vi "Test App.vi"() -> ()   [LabVIEW 2023]
uses:
  typedef/od index.ctl
  xnet_canopen.lvlib
  OD Batch.lvclass
  typedef/Runtime State.ctl
  typedef/NMT State.ctl
  typedef/canopen status formatted.ctl
  <vilib>/Utility/Data Type/Type Definitions/Data Type.ctl
  <vilib>/Utility/Data Type/NI_Data Type.lvlib
panel:
  in  "CAN Interface":refnum<k21>
  out "error out":errorcluster
  out "Write Err":string
  in  "Write Values 2":dbl[](array[numeric])
  in  "Write Values 1":dbl[](array[numeric])
  out "Read Err":string
  out "Read Values 2":T2
  out "Read Values 1":T2
  out "CANOpen Status":T3 {"NMT State" items=["Unknown"=-1, "Initializing"=0, "Pre-Operational"=127, "Operational"=5, "Stopped"=4, "?"=255]; "can_error_status" format="%.0x"}
  in  "Stop":bool
  in  "Start":bool
  in  "Write Batch 2":T6[](array[typedef]) {"SubIndex" format="%.0x"; "Index" format="%.0x"}
  in  "Write Batch 1":T6[](array[typedef]) {"SubIndex" format="%.0x"; "Index" format="%.0x"}
  in  "Read Batch 2":T6[](array[typedef]) {"SubIndex" format="%.0x"; "Index" format="%.0x"}
  in  "Read Batch 1":T6[](array[typedef]) {"SubIndex" format="%.0x"; "Index" format="%.0x"}
  in  "CANOpen LSS Persistence JSON":path
  in  "CANOpen Model JSON":path
  # "Step 1: specify model json and LSS json, \nLSS json will be created if not exists."
  # "Step 3: start if step 1 & 2 are finished."
  # "Step 2: specify Batches to read and write"
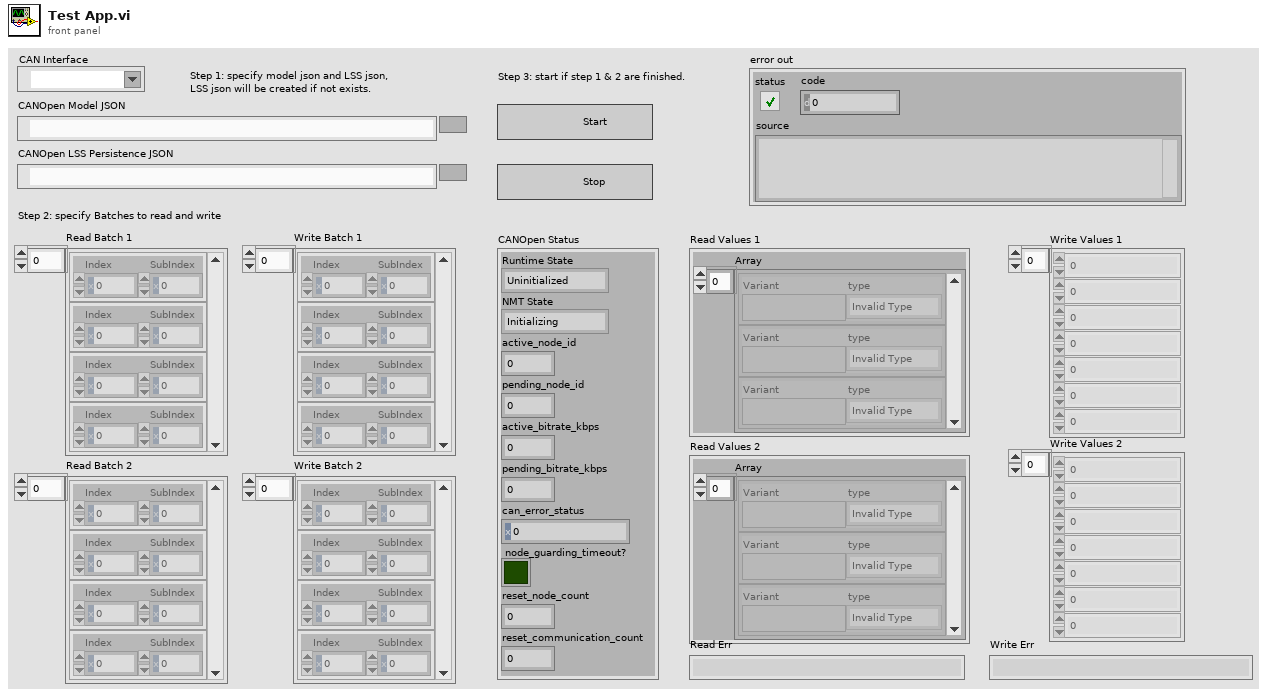
[diagram p1: front panel]
types:
  T1 = typedef "NI_Data Type.lvlib/Data Type.ctl" = enum8{"Invalid Type", "Void", "I8", "I16", "I32", "I64", "U8", "U16", "U32", "U64", "Single Float", "Double Float", "Extended Float", "Single Complex", "Double Complex", "Extended Complex", "Enum U8", "Enum U16", "Enum U32", "Enum U64", "Single Float With Unit", "Double Float With Unit", "Extended Float With Unit", "Single Complex with Unit", "Double Complex with Unit", "Extended Complex with Unit", "Boolean", "String", "Path", "Picture", "Tag", "Array", "Cluster", "Variant", "LV Variant", "Waveform", "Timestamp", "Digital Waveform", "Digital Data", "ExpressData", "Refnum", "External Data", "VI", "Poly VI", "LabVIEW Class Instance", "Fixed Point", "Set Collection", "Map Collection"}
  T2 = cluster{"Array":cluster{"Variant":variant, "type":T1}[]}
  T3 = typedef "xnet_canopen.lvlib/canopen status formatted.ctl" = cluster{"Runtime State":T4, "NMT State":T5, "active_node_id":u32, "pending_node_id":u32, "active_bitrate_kbps":u32, "pending_bitrate_kbps":u32, "can_error_status":u32, "node_guarding_timeout?":bool, "reset_node_count":u32, "reset_communication_count":u32}
  T4 = typedef "xnet_canopen.lvlib/Runtime State.ctl" = enum16{"Uninitialized", "Stopped", "Running", "Failed", "?"}
  T5 = typedef "xnet_canopen.lvlib/NMT State.ctl" = i32
  T6 = typedef "xnet_canopen.lvlib/od index.ctl" = cluster{"Index":u16, "SubIndex":u8}
  T7 = enum8{"Enabled", "Disabled", "Disabled and Grayed Out"}
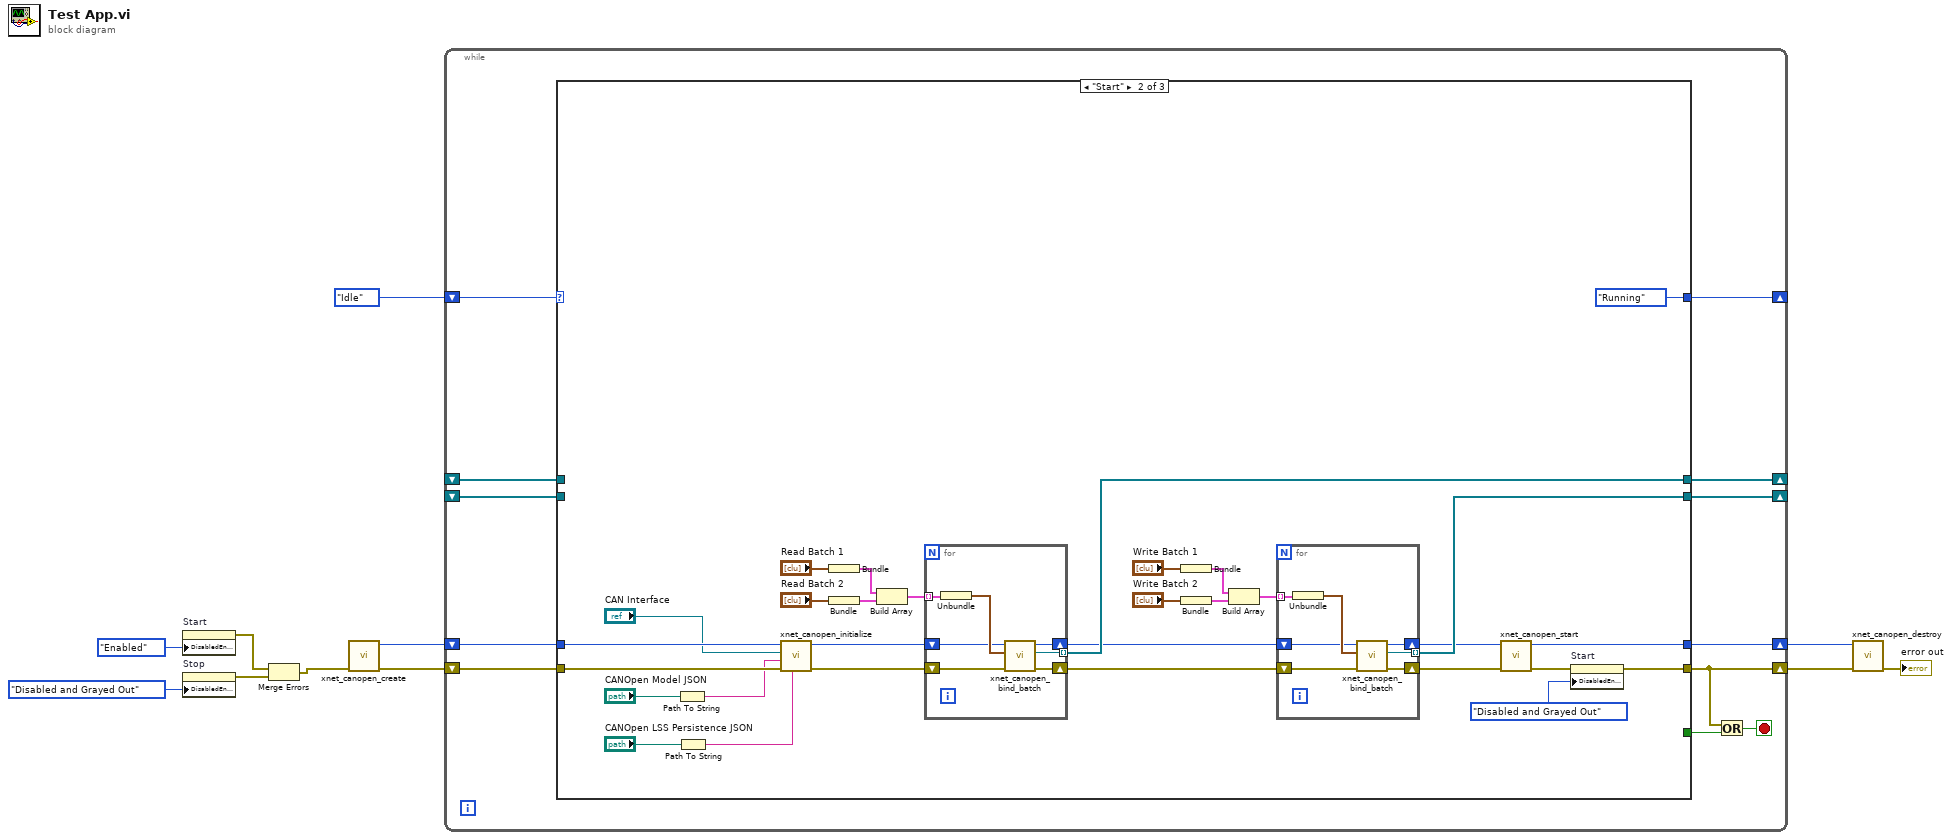
[diagram p0: block diagram]
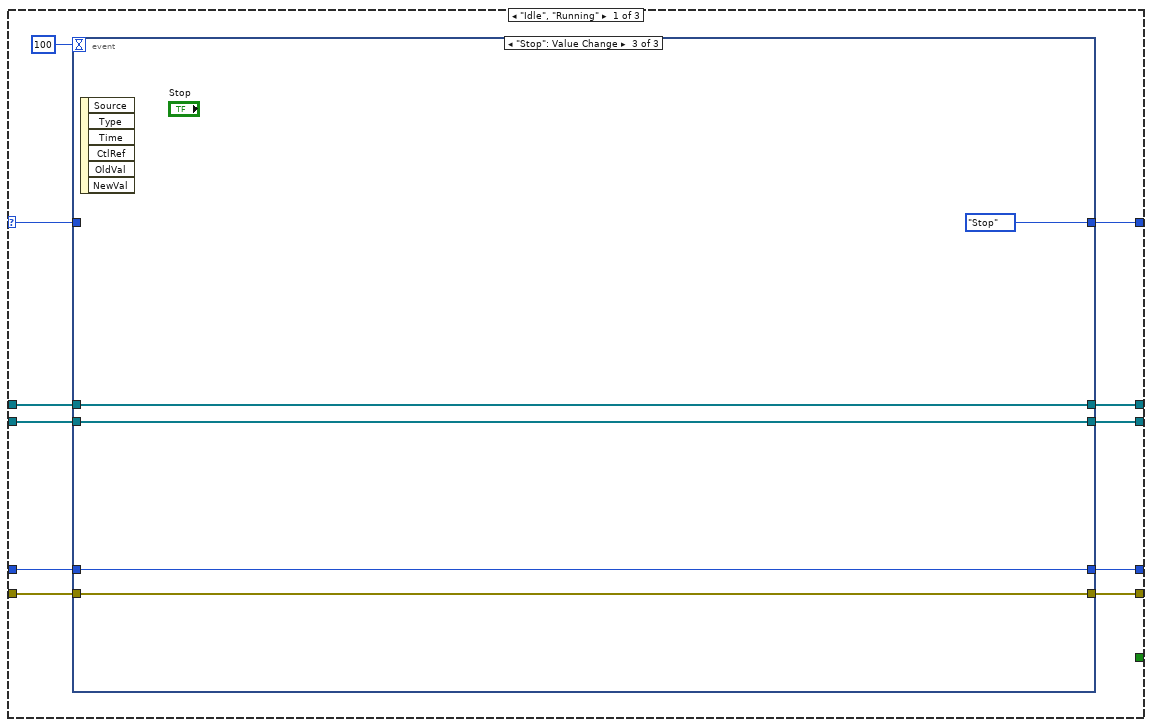
[diagram p2: hidden frame]
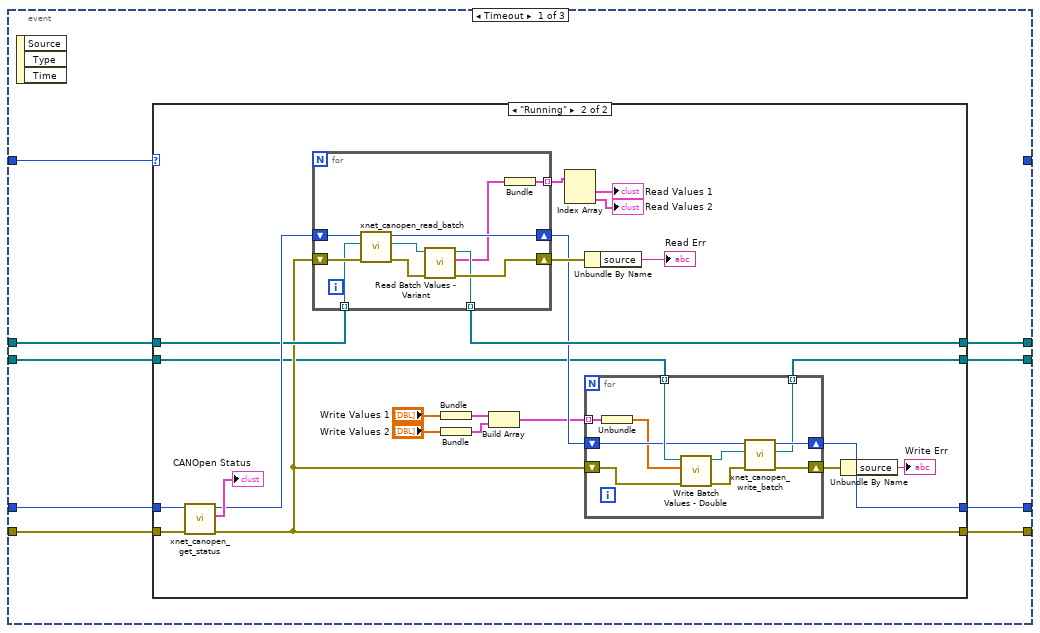
[diagram p3: hidden frame]
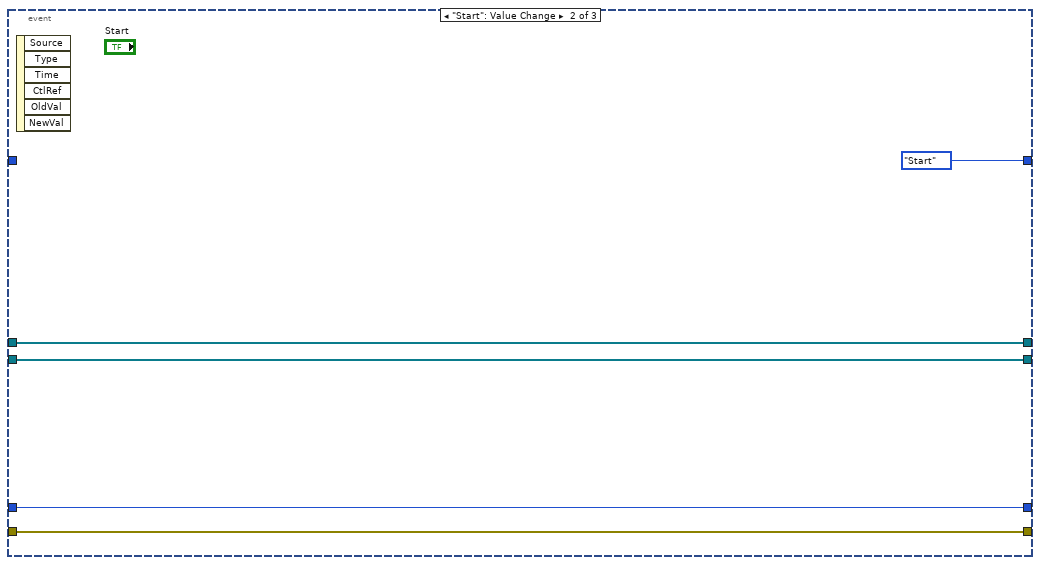
[diagram p5: hidden frame]
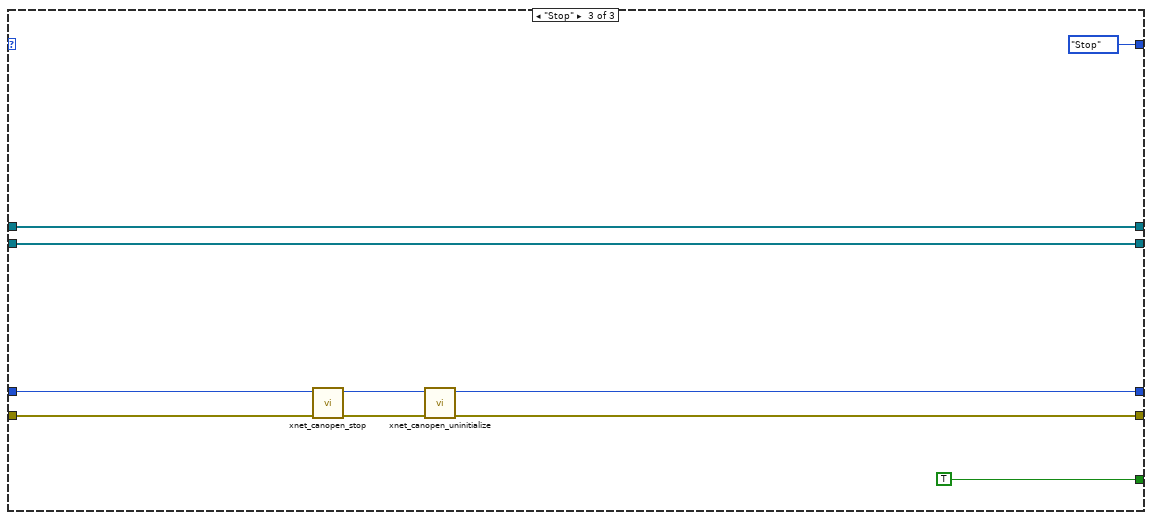
[diagram p6: hidden frame]
diagram:
  n1 = property on="Start" class="Bool"("DisabledEnum"=T7."Enabled" ("Disabled")) -> (error out=w4:errorcluster)  [unwired: 2 in, 1 out]
  n2 = property on="Stop" class="Bool"("DisabledEnum"=T7."Disabled and Grayed Out" ("Disabled")) -> (error out=w2:errorcluster)  [unwired: 2 in, 1 out]
  n3 = Merge Errors(w4, w2) -> (w3:errorcluster)
  n4 = call "xnet_canopen_create.vi"("error in (no error)"=w3) -> ("error out"=w9:errorcluster, "xnet_co_handle"=w10:u64)  [unwired: 9 in]
  n5 = while {
    shift-right: [w23] -> w11
    shift-left: w10 -> [w22]
    shift-right: [w15] -> w8
    shift-left: w9 -> [w21]
    shift-right: [w19] -> _
    shift-left: _ -> [w18]
    shift-right: [w17] -> _
    shift-left: _ -> [w16]
    shift-right: [w12] -> _
    shift-left: enum16{"Idle", "Running", "Start", "Stop"}."Idle" -> [w20]
    stop <- w14 stop-if-true
    n6 = case shown="\"Start\"" w20 {
      selector: w20 -> [w30 _ _]
      tunnel: [w31 w113 w145] -> w23
      tunnel: w22 -> [w32 w107 w151]
      tunnel: w21 -> [w34 w125 w150]
      tunnel: [w33 w110 w147] -> w15
      tunnel: [w28 w124 w154] -> w19
      tunnel: w18 -> [w29 _ w154]
      tunnel: [w26 w116 w153] -> w17
      tunnel: w16 -> [w27 _ w153]
      tunnel: [_ _ TRUE] -> w13
      tunnel: [w24 enum16{"Idle", "Running", "Start", "Stop"}."Running" enum16{"Idle", "Running", "Start", "Stop"}."Stop"] -> w12
      frame "Idle", "Running" {
        n7 = event shown="[2] \"Stop\": Value Change" {
          selector: _ -> [_ _ _]
          dyn-events: _ -> [_ _ _]
          timeout: 100 -> [_ _ _]
          tunnel: w34 -> [w43 w92 w97]
          tunnel: [w42 w92 w97] -> w33
          tunnel: w32 -> [w41 w93 w98]
          tunnel: [w40 w93 w98] -> w31
          tunnel: w30 -> [w39 _ _]
          tunnel: w29 -> [w38 w95 w100]
          tunnel: [w37 w95 w100] -> w28
          tunnel: w27 -> [w36 w94 w99]
          tunnel: [w35 w94 w99] -> w26
          tunnel: [_ enum16{"Idle", "Running", "Start", "Stop"}."Start" enum16{"Idle", "Running", "Start", "Stop"}."Stop"] -> w24
          event Timeout {
            n8 = event-data() -> ()  [unwired: 1 in, 3 out]
            n9 = case shown="\"Running\"" w39 {
              tunnel: w43 -> [w46 w70]
              tunnel: [w46 w57] -> w42
              tunnel: w41 -> [w47 w69]
              tunnel: [w47 w58] -> w40
              tunnel: w38 -> [w45 w66]
              tunnel: [w45 w65] -> w37
              tunnel: w36 -> [w44 w56]
              tunnel: [w44 w55] -> w35
              frame Default {
              }
              frame "Running" {
                n10 = call "xnet_canopen_get_status.vi"("error in (no error)"=w70, "xnet_co_handle_in"=w69) -> ("error out"=w57:errorcluster, "CANOpen Status"=→"CANOpen Status":T3, "xnet_co_handle"=w67:u64)  [unwired: 7 in]
                n11 = for {
                  shift-right: [w85] -> w61
                  shift-left: w57 -> [w90]
                  shift-right: [w87] -> w59
                  shift-left: w67 -> [w88]
                  tunnel: w66 -> [w86] mode=indexing
                  tunnel: [w83] -> w65 mode=indexing
                  tunnel: [w81] -> w64 mode=indexing
                  n12 = call "xnet_canopen_read_batch.vi"("error in (no error)"=w90, "OD Batch in"=w86, "xnet_co_handle_in"=w88) -> ("error out"=w89:errorcluster, "OD Batch"=w84:refnum<class "OD Batch.lvclass">, "xnet_co_handle"=w87:u64)  [unwired: 6 in]
                  n13 = call "Read Batch Values - Variant.vi"("error in (no error)"=w89, "OD Batch in"=w84) -> ("error out"=w85:errorcluster, "Array"=w82:cluster{"Variant":variant, "type":T1}[], "OD Batch out"=w83:refnum<class "OD Batch.lvclass">)  [unwired: 7 in]
                  n14 = Bundle("Array"=w82) -> (w81:T2)  [unwired: 1 in]
                }
                n15 = Bundle("Write Values 1"="Write Values 1") -> (w52:cluster{"Write Values 1":dbl[]})  [unwired: 1 in]
                n16 = Bundle("Write Values 2"="Write Values 2") -> (w51:cluster{"Write Values 2":dbl[]})  [unwired: 1 in]
                n17 = Build Array(w52, w51) -> (w50:cluster{"Write Values 2":dbl[]}[])
                n18 = Index Array(array=w64) -> (element #1=→"Read Values 1":T2, element #2=→"Read Values 2":T2)  [unwired: 2 in]
                n19 = Unbundle By Name(w61) -> ("source"=→"Read Err":string)
                n20 = for {
                  shift-right: [w77] -> w49
                  shift-left: w57 -> [w80]
                  shift-right: [w75] -> w58
                  shift-left: w59 -> [w76]
                  tunnel: [w73] -> w55 mode=indexing
                  tunnel: w56 -> [w78] mode=indexing
                  tunnel: w50 -> [w72] mode=indexing
                  n21 = Unbundle(w72) -> ("Write Values 2"=w71:dbl[])
                  n22 = call "Write Batch Values - Double.vi"("error in (no error)"=w80, "Array"=w71, "OD Batch in"=w78) -> ("error out"=w79:errorcluster, "OD Batch out"=w74:refnum<class "OD Batch.lvclass">)  [unwired: 7 in]
                  n23 = call "xnet_canopen_write_batch.vi"("error in (no error)"=w79, "OD Batch in"=w74, "xnet_co_handle_in"=w76) -> ("error out"=w77:errorcluster, "OD Batch"=w73:refnum<class "OD Batch.lvclass">, "xnet_co_handle"=w75:u64)  [unwired: 6 in]
                }
                n24 = Unbundle By Name(w49) -> ("source"=→"Write Err":string)
              }
            }
          }
          event "Start": Value Change {
            n25 = event-data() -> ()  [unwired: 1 in, 6 out]
          }
          event "Stop": Value Change {
            n26 = event-data() -> ()  [unwired: 1 in, 6 out]
          }
        }
      }
      frame "Start" {
        n27 = Path To String(path="CANOpen Model JSON") -> (string=w102:string)
        n28 = Path To String(path="CANOpen LSS Persistence JSON") -> (string=w101:string)
        n29 = call "xnet_canopen_initialize.vi"("persistence LSS path"=w101, "error in (no error)"=w125, "model json path"=w102, "XNET Interface"="CAN Interface", "xnet_co_handle_in"=w107) -> ("error out"=w108:errorcluster, "xnet_co_handle"=w106:u64)  [unwired: 5 in]
        n30 = Bundle("Read Batch 1"="Read Batch 1") -> (w128:cluster{"Read Batch 1":T6[]})  [unwired: 1 in]
        n31 = Bundle("Read Batch 2"="Read Batch 2") -> (w127:cluster{"Read Batch 2":T6[]})  [unwired: 1 in]
        n32 = Build Array(w128, w127) -> (w126:cluster{"Read Batch 2":T6[]}[])
        n33 = for {
          tunnel: w126 -> [w144] mode=indexing
          tunnel: [w140] -> w124 mode=indexing
          shift-right: [w139] -> w123
          shift-left: w106 -> [w142]
          shift-right: [w138] -> w122
          shift-left: w108 -> [w141]
          n34 = Unbundle(w144) -> ("Read Batch 2"=w143:T6[])
          n35 = call "xnet_canopen_bind_batch.vi"("error in (no error)"=w141, "OD Indices"=w143, "xnet_co_handle_in"=w142) -> ("error out"=w138:errorcluster, "OD Batch"=w140:refnum<class "OD Batch.lvclass">, "xnet_co_handle"=w139:u64)  [unwired: 6 in]
        }
        n36 = Bundle("Write Batch 1"="Write Batch 1") -> (w121:cluster{"Write Batch 1":T6[]})  [unwired: 1 in]
        n37 = Bundle("Write Batch 2"="Write Batch 2") -> (w120:cluster{"Write Batch 2":T6[]})  [unwired: 1 in]
        n38 = Build Array(w121, w120) -> (w119:cluster{"Write Batch 2":T6[]}[])
        n39 = for {
          tunnel: w119 -> [w137] mode=indexing
          tunnel: [w134] -> w116 mode=indexing
          shift-right: [w132] -> w114
          shift-left: w123 -> [w135]
          shift-right: [w131] -> w115
          shift-left: w122 -> [w133]
          n40 = Unbundle(w137) -> ("Write Batch 2"=w136:T6[])
          n41 = call "xnet_canopen_bind_batch.vi"("error in (no error)"=w133, "OD Indices"=w136, "xnet_co_handle_in"=w135) -> ("error out"=w131:errorcluster, "OD Batch"=w134:refnum<class "OD Batch.lvclass">, "xnet_co_handle"=w132:u64)  [unwired: 6 in]
        }
        n42 = call "xnet_canopen_start.vi"("error in (no error)"=w115, "xnet_co_handle_in"=w114) -> ("error out"=w111:errorcluster, "xnet_co_handle"=w113:u64)  [unwired: 8 in]
        n43 = property on="Start" class="Bool"(error in=w111, "DisabledEnum"=T7."Disabled and Grayed Out" ("Disabled")) -> (error out=w110:errorcluster)  [unwired: 1 in, 1 out]
      }
      frame "Stop" {
        n44 = call "xnet_canopen_stop.vi"("error in (no error)"=w150, "xnet_co_handle_in"=w151) -> ("error out"=w152:errorcluster, "xnet_co_handle"=w146:u64)  [unwired: 8 in]
        n45 = call "xnet_canopen_uninitialize.vi"("error in (no error)"=w152, "xnet_co_handle_in"=w146) -> ("error out"=w147:errorcluster, "xnet_co_handle"=w145:u64)  [unwired: 8 in]
      }
    }
    n46 = Or(x=w15, y=w13) -> (x .or. y?=w14:bool)
  }
  n47 = call "xnet_canopen_destroy.vi"("error in (no error)"=w8, "xnet_co_handle"=w11) -> ("error out"=→"error out":errorcluster)  [unwired: 9 in]
